vi "fake tool picture outputs.vi"(10 "start":timestamp, 11 "text":string) -> (0 "mode":enum16{"slow", "fast"}(ring), 1 "time":timestamp, 2 "label":string, 3 "count":i32, 4 "picture":picture)   [LabVIEW 2020, in "MCP Server tests.lvlib"]
doc: "Fake tool to test structured output: ordinary outputs of several types (I32, string, timestamp, U16 enum) next to a picture output. tools/call must return the ordinary outputs in structuredContent and in the text, the picture as a separate image item, and tools/list must give an outputSchema without the picture."
uses:
  MCP Server tests.lvlib
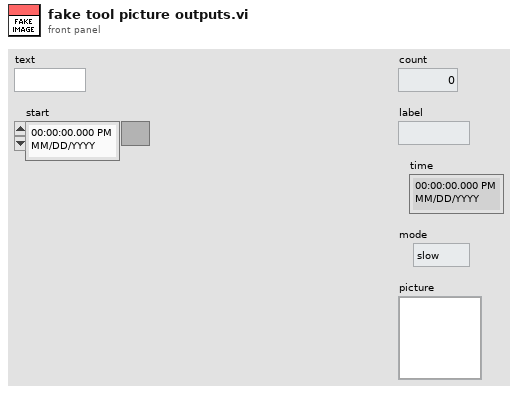
[diagram p1: front panel]
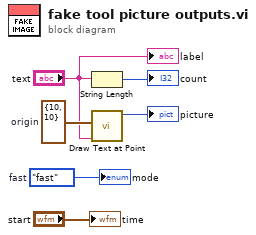
[diagram p0: block diagram]
diagram:
  w6 = cluster{"x":i16, "y":i16} {"x"=10, "y"=10}  # origin
  w2 = enum16{"slow", "fast"}."fast"  # fast
  n1 = String Length(string="text") -> (length=→"count":i32)
  n2 = call <vilib>:"Draw Text at Point.vi"("text"="text", "origin"=w6) -> ("new picture"=→"picture":picture)  [unwired: 8 in, 1 out]
  "label" <- "text"
  "time" <- "start"
  "mode" <- w2
